vi "HandleItemActivation.vi"(8 "error in (no error)":errorcluster, 11 "GettingStartedWindow.lvlib:Manual.lvclass":refnum<class "Manual.lvclass">) -> (0 "error out":errorcluster, 3 "GettingStartedWindow.lvlib:Manual.lvclass 2":refnum<class "Manual.lvclass">)   [LabVIEW 2023, in "GettingStartedWindow.lvlib" / "Manual.lvclass"]
uses:
  <resource>/modes/FRC/Classes/Manual/Manual.lvclass
  <resource>/modes/FRC/Classes/Manual/Manual.lvclass/Manual.ctl
  <resource>/modes/FRC/LocalizedStrings.vi
  <vilib>/Platform/browser.llb/Open Acrobat Document.vi
  <resource>/modes/FRC/GettingStartedWindow.lvlib
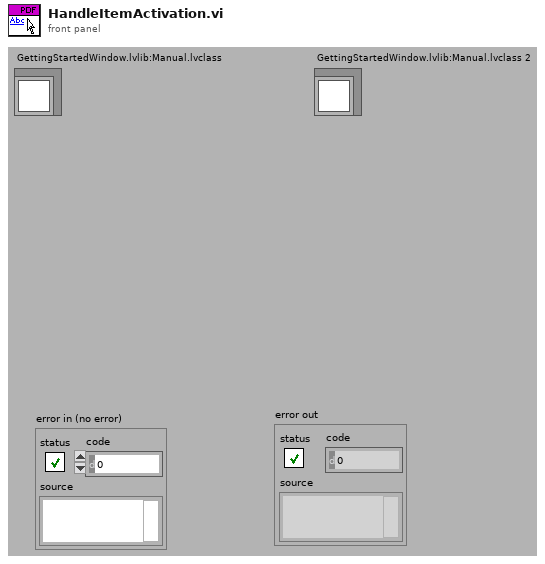
[diagram p1: front panel]
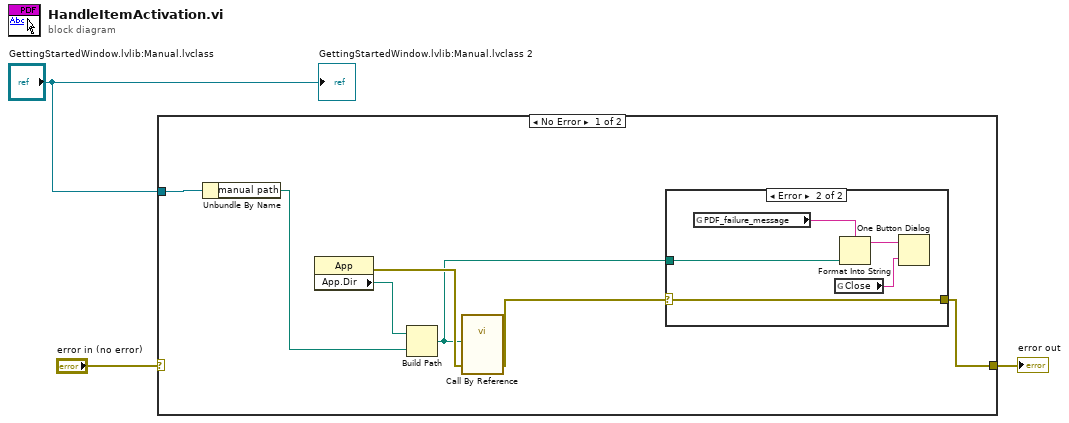
[diagram p0: block diagram]
diagram:
  n1 = case shown="No Error" "error in (no error)" {
    selector: "error in (no error)" -> [_ w17]
    tunnel: [w6 w17] -> w2
    tunnel: "GettingStartedWindow.lvlib:Manual.lvclass" -> [w8 _]
    frame No Error {
      n2 = Unbundle By Name(w8) -> ("manual path"=w7:path)
      n3 = property class="App"() -> (error out=w9:errorcluster, "App.Dir"=w10:path)  [unwired: 2 in, 1 out]
      n4 = Build Path(base path=w10, name or relative path=w7) -> (appended path=w5:path)
      n5 = call-by-ref "?"("error in (no error)"=w9, "acrobat document"=w5) -> ("error out"=w4:errorcluster)  [unwired: 2 in, 7 out]
      n6 = case shown="Error" w4 {
        selector: w4 -> [w11 w16]
        tunnel: [w11 w16] -> w6
        tunnel: w5 -> [_ w15]
        frame No Error {
        }
        frame Error {
          n7 = global read "LocalizedStrings.vi" "PDF_failure_message"() -> (w13:string)
          n8 = global read "LocalizedStrings.vi" "Close"() -> (w12:string)
          n9 = Format Into String(format string=w13, w15) -> (resulting string=w14:string)  [unwired: 2 in, 1 out]
          n10 = One Button Dialog(message=w14, button name ("OK")=w12) -> ()  [unwired: 1 out]
        }
      }
    }
    frame Error {
    }
  }
  "error out" <- w2
  "GettingStartedWindow.lvlib:Manual.lvclass 2" <- "GettingStartedWindow.lvlib:Manual.lvclass"
